vi "LaneFolower.vi"() -> ()   [LabVIEW 2024]
uses:
  <vilib>/Python/Open Venv Python Session.vi
panel:
  in  "File Path":path
  out "Image":T1(plugin-control)
  in  "Lane_No.":i32
  out "ToGoLane_X":dbl[](array[numeric])=[-0.07318960875272751, -0.07601258158683777, -0.07903728634119034, -0.08227015286684036, -0.08571790158748627, -0.08938748389482498, -0.09328625351190567, -0.09742185473442078, -0.1018022671341896, -0.10643591731786728, -0.11133154481649399, -0.11649835854768753, -0.12194599956274033, -0.1276845932006836, -0.13372473418712616, -0.140077605843544, -0.1467549204826355, -0.15376901626586914, -0.1611328274011612, -0.16886006295681, -0.17696507275104523, -0.18546302616596222, -0.19436998665332794, -0.20370280742645264, -0.2134794145822525, -0.22371862828731537, -0.23444052040576935, -0.2456662356853485, -0.2574182152748108, -0.26972031593322754, -0.2825978398323059, -0.2960776686668396, -0.3101884424686432, -0.3249606192111969, -0.3404266834259033, -0.35662132501602173, -0.3735816180706024, -0.39134714007377625, -0.4099603295326233, -0.4294666647911072, -0.44991496205329895, -0.47135770320892334, -0.49385130405426025, -0.5174566507339478, -0.5422393083572388, -0.5682703852653503, -0.5956265330314636, -0.6243910789489746, -0.6546544432640076, -0.6865149736404419]
  out "ToGpLane_Y":dbl[](array[numeric])=[0.040495745837688446, 0.047222185879945755, 0.05409690737724304, 0.06112465262413025, 0.06831060349941254, 0.07565993815660477, 0.08317827433347702, 0.09087134152650833, 0.09874525666236877, 0.10680633038282394, 0.1150611862540245, 0.12351679056882858, 0.13218039274215698, 0.14105971157550812, 0.1501627415418625, 0.159497931599617, 0.16907407343387604, 0.1789005994796753, 0.18898724019527435, 0.19934435188770294, 0.20998279750347137, 0.22091402113437653, 0.23215018212795258, 0.24370405077934265, 0.2555891275405884, 0.2678196132183075, 0.2804107666015625, 0.2933785319328308, 0.306739866733551, 0.3205127418041229, 0.3347163796424866, 0.349371075630188, 0.36449843645095825, 0.38012149930000305, 0.3962647616863251, 0.41295456886291504, 0.43021881580352783, 0.4480874836444855, 0.46659258008003235, 0.48576855659484863, 0.5056522488594055, 0.526283323764801, 0.5477043986320496, 0.5699615478515625, 0.5931042432785034, 0.6171862483024597, 0.6422654986381531, 0.6684049367904663, 0.6956729292869568, 0.7241437435150146]
  out "Tracking_Err(m)":dbl=0.08364582631744388
  in  "Ld(m)":dbl=1.0 format="%#_13g"
  out "GPS_Steer_CMD(Deg)":dbl=-20.0
  out "Lane":T2(graph)=[{"Third_Lane_X"=[-0.07318960875272751, -0.07601258158683777, -0.07903728634119034, -0.08227015286684036, -0.08571790158748627, -0.08938748389482498, -0.09328625351190567, -0.09742185473442078, -0.1018022671341896, -0.10643591731786728, -0.11133154481649399, -0.11649835854768753, -0.12194599956274033, -0.1276845932006836, -0.13372473418712616, -0.140077605843544, -0.1467549204826355, -0.15376901626586914, -0.1611328274011612, -0.16886006295681, -0.17696507275104523, -0.18546302616596222, -0.19436998665332794, -0.20370280742645264, -0.2134794145822525, -0.22371862828731537, -0.23444052040576935, -0.2456662356853485, -0.2574182152748108, -0.26972031593322754, -0.2825978398323059, -0.2960776686668396, -0.3101884424686432, -0.3249606192111969, -0.3404266834259033, -0.35662132501602173, -0.3735816180706024, -0.39134714007377625, -0.4099603295326233, -0.4294666647911072, -0.44991496205329895, -0.47135770320892334, -0.49385130405426025, -0.5174566507339478, -0.5422393083572388, -0.5682703852653503, -0.5956265330314636, -0.6243910789489746, -0.6546544432640076, -0.6865149736404419], "Third_Lane_Y"=[0.040495745837688446, 0.047222185879945755, 0.05409690737724304, 0.06112465262413025, 0.06831060349941254, 0.07565993815660477, 0.08317827433347702, 0.09087134152650833, 0.09874525666236877, 0.10680633038282394, 0.1150611862540245, 0.12351679056882858, 0.13218039274215698, 0.14105971157550812, 0.1501627415418625, 0.159497931599617, 0.16907407343387604, 0.1789005994796753, 0.18898724019527435, 0.19934435188770294, 0.20998279750347137, 0.22091402113437653, 0.23215018212795258, 0.24370405077934265, 0.2555891275405884, 0.2678196132183075, 0.2804107666015625, 0.2933785319328308, 0.306739866733551, 0.3205127418041229, 0.3347163796424866, 0.349371075630188, 0.36449843645095825, 0.38012149930000305, 0.3962647616863251, 0.41295456886291504, 0.43021881580352783, 0.4480874836444855, 0.46659258008003235, 0.48576855659484863, 0.5056522488594055, 0.526283323764801, 0.5477043986320496, 0.5699615478515625, 0.5931042432785034, 0.6171862483024597, 0.6422654986381531, 0.6684049367904663, 0.6956729292869568, 0.7241437435150146]}, {"Third_Lane_X"=[0.3850393295288086, 0.38269442319869995, 0.3802776634693146, 0.37778156995773315, 0.37519851326942444, 0.37252023816108704, 0.36973854899406433, 0.3668445944786072, 0.36382946372032166, 0.3606834411621094, 0.3573968708515167, 0.35395947098731995, 0.3503605127334595, 0.3465888500213623, 0.34263283014297485, 0.3384802043437958, 0.33411839604377747, 0.3295340836048126, 0.3247132897377014, 0.31964147090911865, 0.3143034875392914, 0.3086833655834198, 0.30276429653167725, 0.29652881622314453, 0.2899583876132965, 0.2830337584018707, 0.2757345139980316, 0.2680392861366272, 0.2599255442619324, 0.25136950612068176, 0.24234625697135925, 0.23282931745052338, 0.22279086709022522, 0.21220147609710693, 0.201029971241951, 0.1892433911561966, 0.17680683732032776, 0.16368332505226135, 0.14983347058296204, 0.135215625166893, 0.1197853684425354, 0.10349543392658234, 0.0862954780459404, 0.06813178956508636, 0.048946939408779144, 0.028679724782705307, 0.007264426909387112, -0.015369318425655365, -0.03929702565073967, -0.06459984183311462], "Third_Lane_Y"=[0.07649079710245132, 0.08298972249031067, 0.08961328864097595, 0.09636534750461578, 0.10325001180171967, 0.11027147620916367, 0.11743411421775818, 0.12474247813224792, 0.1322014033794403, 0.1398158222436905, 0.14759093523025513, 0.155532106757164, 0.16364507377147675, 0.17193572223186493, 0.180410236120224, 0.18907500803470612, 0.19793690741062164, 0.20700296759605408, 0.21628059446811676, 0.2257775366306305, 0.23550201952457428, 0.2454625517129898, 0.25566813349723816, 0.2661281228065491, 0.276852548122406, 0.28785181045532227, 0.29913684725761414, 0.31071919202804565, 0.32261112332344055, 0.33482545614242554, 0.3473757207393646, 0.3602762222290039, 0.3735422194004059, 0.387189656496048, 0.4012354910373688, 0.4156976342201233, 0.4305952489376068, 0.4459485411643982, 0.4617789089679718, 0.4781092703342438, 0.4949638843536377, 0.5123687386512756, 0.5303513407707214, 0.5489413142204285, 0.5681700706481934, 0.5880714654922485, 0.6086814403533936, 0.6300389170646667, 0.6521854400634766, 0.6751657128334045]}, {"Third_Lane_X"=[0.0, 0.0, 0.0, 0.0, 0.0, 0.0, 0.0, 0.0, 0.0, 0.0, 0.0, 0.0, 0.0, 0.0, 0.0, 0.0, 0.0, 0.0, 0.0, 0.0, 0.0, 0.0, 0.0, 0.0, 0.0, 0.0, 0.0, 0.0, 0.0, 0.0, 0.0, 0.0, 0.0, 0.0, 0.0, 0.0, 0.0, 0.0, 0.0, 0.0, 0.0, 0.0, 0.0, 0.0, 0.0, 0.0, 0.0, 0.0, 0.0, 0.0], "Third_Lane_Y"=[0.0, 0.0, 0.0, 0.0, 0.0, 0.0, 0.0, 0.0, 0.0, 0.0, 0.0, 0.0, 0.0, 0.0, 0.0, 0.0, 0.0, 0.0, 0.0, 0.0, 0.0, 0.0, 0.0, 0.0, 0.0, 0.0, 0.0, 0.0, 0.0, 0.0, 0.0, 0.0, 0.0, 0.0, 0.0, 0.0, 0.0, 0.0, 0.0, 0.0, 0.0, 0.0, 0.0, 0.0, 0.0, 0.0, 0.0, 0.0, 0.0, 0.0]}]
  out "Third_Lane_X":dbl[](array[numeric])
  out "Third_Lane_Y":dbl[](array[numeric])
  out "Second_Lane_X":dbl[](array[numeric])=[0.3850393295288086, 0.38269442319869995, 0.3802776634693146, 0.37778156995773315, 0.37519851326942444, 0.37252023816108704, 0.36973854899406433, 0.3668445944786072, 0.36382946372032166, 0.3606834411621094, 0.3573968708515167, 0.35395947098731995, 0.3503605127334595, 0.3465888500213623, 0.34263283014297485, 0.3384802043437958, 0.33411839604377747, 0.3295340836048126, 0.3247132897377014, 0.31964147090911865, 0.3143034875392914, 0.3086833655834198, 0.30276429653167725, 0.29652881622314453, 0.2899583876132965, 0.2830337584018707, 0.2757345139980316, 0.2680392861366272, 0.2599255442619324, 0.25136950612068176, 0.24234625697135925, 0.23282931745052338, 0.22279086709022522, 0.21220147609710693, 0.201029971241951, 0.1892433911561966, 0.17680683732032776, 0.16368332505226135, 0.14983347058296204, 0.135215625166893, 0.1197853684425354, 0.10349543392658234, 0.0862954780459404, 0.06813178956508636, 0.048946939408779144, 0.028679724782705307, 0.007264426909387112, -0.015369318425655365, -0.03929702565073967, -0.06459984183311462]
  out "Second_Lane_Y":dbl[](array[numeric])=[0.07649079710245132, 0.08298972249031067, 0.08961328864097595, 0.09636534750461578, 0.10325001180171967, 0.11027147620916367, 0.11743411421775818, 0.12474247813224792, 0.1322014033794403, 0.1398158222436905, 0.14759093523025513, 0.155532106757164, 0.16364507377147675, 0.17193572223186493, 0.180410236120224, 0.18907500803470612, 0.19793690741062164, 0.20700296759605408, 0.21628059446811676, 0.2257775366306305, 0.23550201952457428, 0.2454625517129898, 0.25566813349723816, 0.2661281228065491, 0.276852548122406, 0.28785181045532227, 0.29913684725761414, 0.31071919202804565, 0.32261112332344055, 0.33482545614242554, 0.3473757207393646, 0.3602762222290039, 0.3735422194004059, 0.387189656496048, 0.4012354910373688, 0.4156976342201233, 0.4305952489376068, 0.4459485411643982, 0.4617789089679718, 0.4781092703342438, 0.4949638843536377, 0.5123687386512756, 0.5303513407707214, 0.5489413142204285, 0.5681700706481934, 0.5880714654922485, 0.6086814403533936, 0.6300389170646667, 0.6521854400634766, 0.6751657128334045]
  out "First_Lane_Y":dbl[](array[numeric])=[0.040495745837688446, 0.047222185879945755, 0.05409690737724304, 0.06112465262413025, 0.06831060349941254, 0.07565993815660477, 0.08317827433347702, 0.09087134152650833, 0.09874525666236877, 0.10680633038282394, 0.1150611862540245, 0.12351679056882858, 0.13218039274215698, 0.14105971157550812, 0.1501627415418625, 0.159497931599617, 0.16907407343387604, 0.1789005994796753, 0.18898724019527435, 0.19934435188770294, 0.20998279750347137, 0.22091402113437653, 0.23215018212795258, 0.24370405077934265, 0.2555891275405884, 0.2678196132183075, 0.2804107666015625, 0.2933785319328308, 0.306739866733551, 0.3205127418041229, 0.3347163796424866, 0.349371075630188, 0.36449843645095825, 0.38012149930000305, 0.3962647616863251, 0.41295456886291504, 0.43021881580352783, 0.4480874836444855, 0.46659258008003235, 0.48576855659484863, 0.5056522488594055, 0.526283323764801, 0.5477043986320496, 0.5699615478515625, 0.5931042432785034, 0.6171862483024597, 0.6422654986381531, 0.6684049367904663, 0.6956729292869568, 0.7241437435150146]
  out "First_Lane_X":dbl[](array[numeric])=[-0.07318960875272751, -0.07601258158683777, -0.07903728634119034, -0.08227015286684036, -0.08571790158748627, -0.08938748389482498, -0.09328625351190567, -0.09742185473442078, -0.1018022671341896, -0.10643591731786728, -0.11133154481649399, -0.11649835854768753, -0.12194599956274033, -0.1276845932006836, -0.13372473418712616, -0.140077605843544, -0.1467549204826355, -0.15376901626586914, -0.1611328274011612, -0.16886006295681, -0.17696507275104523, -0.18546302616596222, -0.19436998665332794, -0.20370280742645264, -0.2134794145822525, -0.22371862828731537, -0.23444052040576935, -0.2456662356853485, -0.2574182152748108, -0.26972031593322754, -0.2825978398323059, -0.2960776686668396, -0.3101884424686432, -0.3249606192111969, -0.3404266834259033, -0.35662132501602173, -0.3735816180706024, -0.39134714007377625, -0.4099603295326233, -0.4294666647911072, -0.44991496205329895, -0.47135770320892334, -0.49385130405426025, -0.5174566507339478, -0.5422393083572388, -0.5682703852653503, -0.5956265330314636, -0.6243910789489746, -0.6546544432640076, -0.6865149736404419]
  out "error out":errorcluster
  out "Python Loop Process Time":u32=34
  in  "stop":bool
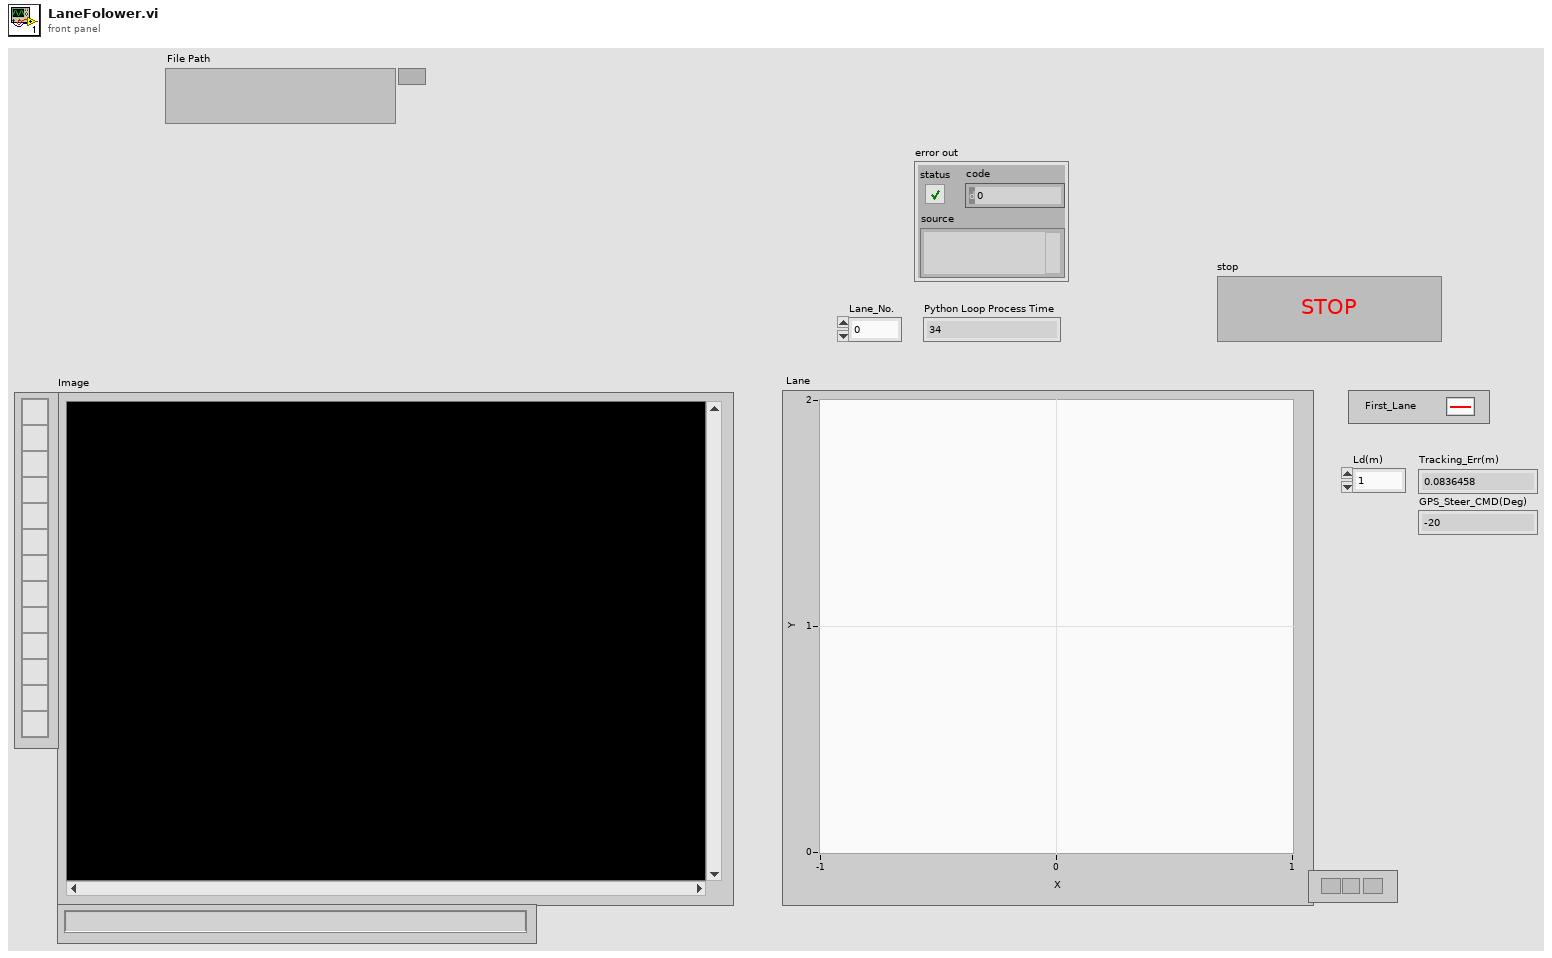
[diagram p1: front panel]
types:
  T1 = typedef "IMAQ Image.ctl" = refnum<image>
  T2 = cluster{"Third_Lane_X":dbl[], "Third_Lane_Y":dbl[]}[]
  T3 = cluster{"First_Lane_X":dbl[], "First_Lane_Y":dbl[]}
  T4 = cluster{"Second_Lane_X":dbl[], "Second_Lane_Y":dbl[]}
  T5 = cluster{"Third_Lane_X":dbl[], "Third_Lane_Y":dbl[]}
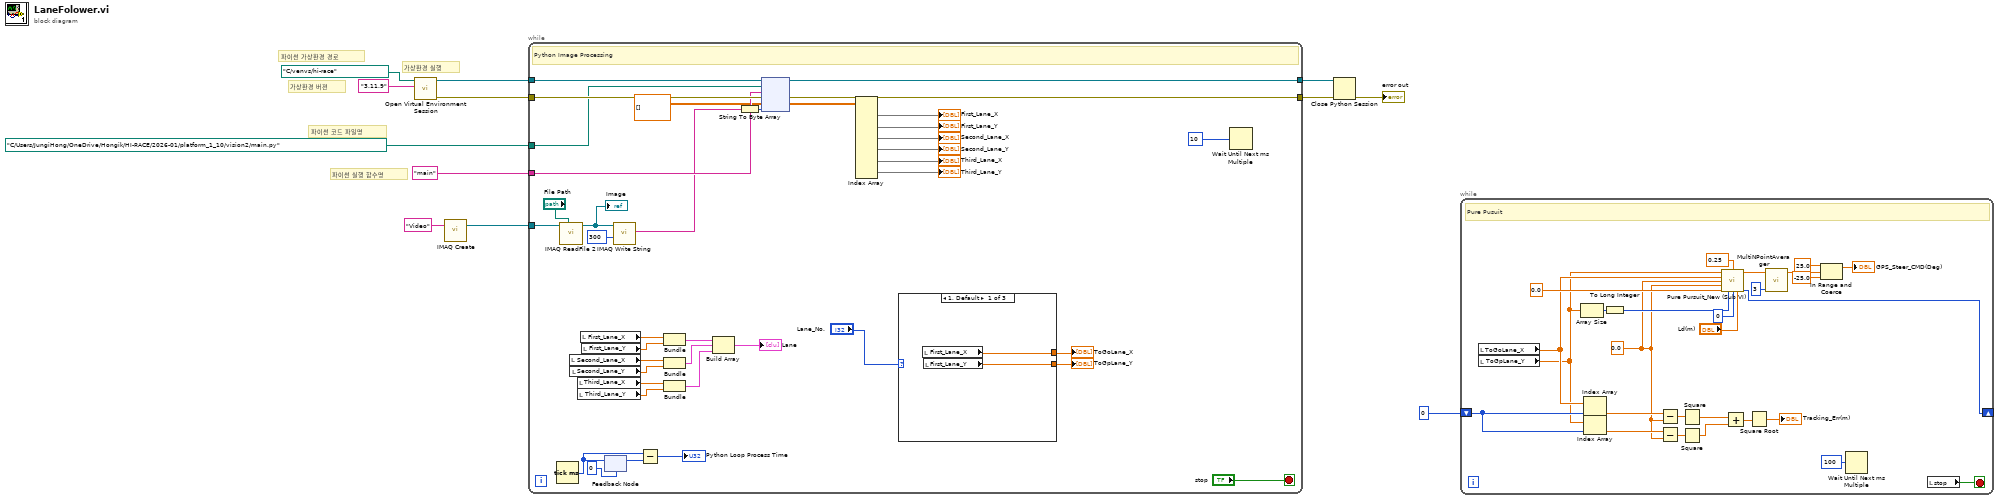
[diagram p0: block diagram]
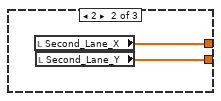
[diagram p2: hidden frame]
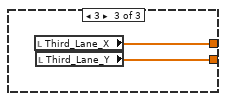
[diagram p3: hidden frame]
diagram:
  # "파이썬 실행 함수명"
  # "파이썬 코드 파일명"
  # "가상환경 실행"
  # "가상환경 버젼"
  # "파이썬 가상환경 경로"
  n1 = call-poly <vilib>:"Open Virtual Environment Session.vi"("Python version"="3.11.9", "Env path"=path "C:/venvs/hi-race") -> ("error out"=w7:errorcluster, "session out"=w8:refnum<k35>)  [unwired: 8 in]
  n2 = call "IMAQ Create"("Image Name"="Video") -> ("New Image"=w1:T1)  [unwired: 4 in, 1 out]
  n3 = while {
    tunnel: path "C:/Users/JungiHong/OneDrive/Hongik/HI-RACE/2026-01/platform_1_10/vision2/main.py" ("Name") -> [w47]
    tunnel: "main" ("module out") -> [w46]
    tunnel: w8 -> [w49]
    tunnel: [w51] -> w10
    tunnel: w7 -> [w48]
    tunnel: [w50] -> w9
    tunnel: w1 -> [w15]
    stop <- "stop" stop-if-true
    # "Python Image Processing"
    n4 = Tick Count (ms)() -> (millisecond timer value=w42:u32)
    n5 = call "IMAQ ReadFile 2"("File Path"="File Path", "Image"=w15) -> ("Image Out"=w14:T1)  [unwired: 5 in, 4 out]
    "Image" <- w14
    n6 = local read "Second_Lane_X"() -> (w32:dbl[])
    n7 = local read "Second_Lane_Y"() -> (w31:dbl[])
    n8 = local read "Third_Lane_X"() -> (w30:dbl[])
    n9 = local read "Third_Lane_Y"() -> (w29:dbl[])
    n10 = local read "First_Lane_X"() -> (w34:dbl[])
    n11 = local read "First_Lane_Y"() -> (w33:dbl[])
    n12 = feedback #1(u32 0 ("millisecond timer value")) -> (w43:u32)
    n13 = feedback-in #1(w42) -> ()
    n14 = call-poly "IMAQ Write String"("Image Quality"=u32 300, "Image"=w14) -> ("FileString"=w16:string)  [unwired: 7 in, 2 out]
    n15 = Subtract(x=w42, y=w43) -> (x-y=→"Python Loop Process Time":u32)
    n16 = Bundle("First_Lane_X"=w34, "First_Lane_Y"=w33) -> (w28:T3)  [unwired: 1 in]
    n17 = Bundle("Second_Lane_X"=w32, "Second_Lane_Y"=w31) -> (w27:T4)  [unwired: 1 in]
    n18 = Bundle("Third_Lane_X"=w30, "Third_Lane_Y"=w29) -> (w26:T5)  [unwired: 1 in]
    n19 = Build Array(w28, w27, w26) -> (→"Lane":T2)
    n20 = String To Byte Array(string=w16) -> (unsigned byte array=w41:u8[])
    n21 = node(w49, w47, w46, w48, dbl[][] [] ("appended array"), w41) -> (w51:refnum<k35>, w50:errorcluster, w20:dbl[][])  [unwired: 1 in, 2 out]
    n22 = Index Array(array=w20) -> (element #1=→"First_Lane_X":dbl[], element #2=→"First_Lane_Y":dbl[], element #3=→"Second_Lane_X":dbl[], element #4=→"Second_Lane_Y":dbl[], element #5=→"Third_Lane_X":dbl[], element #6=→"Third_Lane_Y":dbl[])  [unwired: 12 in]
    n23 = case shown="1, Default" "Lane_No." {
      tunnel: [w53 w55 w57] -> w23
      tunnel: [w52 w54 w56] -> w22
      frame 1, Default {
        n24 = local read "First_Lane_X"() -> (w53:dbl[])
        n25 = local read "First_Lane_Y"() -> (w52:dbl[])
      }
      frame 2 {
        n26 = local read "Second_Lane_X"() -> (w55:dbl[])
        n27 = local read "Second_Lane_Y"() -> (w54:dbl[])
      }
      frame 3 {
        n28 = local read "Third_Lane_X"() -> (w57:dbl[])
        n29 = local read "Third_Lane_Y"() -> (w56:dbl[])
      }
    }
    "ToGoLane_X" <- w23
    "ToGpLane_Y" <- w22
    n30 = Wait Until Next ms Multiple(millisecond multiple=u32 10) -> ()  [unwired: 1 out]
  }
  n31 = Close Python Session(session in=w10, error in=w9) -> (11:→"error out":errorcluster)
  n32 = while {
    shift-right: [w84] -> _
    shift-left: 0 ("Index(near vehicle)") -> [w83]
    stop <- w82 stop-if-true
    w58 = 0.0 ("Y_Current")
    # "Pure Pusuit"
    n33 = local read "ToGoLane_X"() -> (w60:dbl[])
    n34 = local read "ToGpLane_Y"() -> (w59:dbl[])
    n35 = Array Size(array=w59) -> (size(s)=w69:i32)
    n36 = Index Array(array=w60, index=w83) -> (element=w80:dbl)
    n37 = Index Array(array=w59, index=w83) -> (element=w81:dbl)
    n38 = To Long Integer(number=w69) -> (32bit integer=w68:i32)
    n39 = Subtract(x=w80, y=w58) -> (x-y=w75:dbl)
    n40 = Subtract(x=w81, y=w58) -> (x-y=w74:dbl)
    n41 = Square(x=w75) -> (x^2=w73:dbl)
    n42 = Square(x=w74) -> (x^2=w72:dbl)
    n43 = call "Pure Pursuit_New (Sub VI).vi"("x_lat_path"=w59, "L"=0.25, "y_long_path"=w60, "X_Current"=w58, "Y_Current"=w58, "Heading_Current"=0.0, "#pnt"=w68, "WP no_pre"=0, "LAD"="Ld(m)") -> ("Steer_CMD(Deg)"=w64:dbl, "Index(near vehicle)"=w84:i32)  [unwired: 3 in, 2 out]
    n44 = Add(x=w73, y=w72) -> (x+y=w71:dbl)
    n45 = Square Root(x=w71) -> (sqrt(x)=→"Tracking_Err(m)":dbl)
    n46 = call "MultiNPointAverager.vi"("N point average"=3 ("WP no_pre"), "Data_input"=w64) -> ("숫자형"=w79:dbl)  [unwired: 9 in]
    n47 = In Range and Coerce(upper limit=25.0, x=w79, lower limit=-25.0) -> (coerced(x)=→"GPS_Steer_CMD(Deg)":dbl)  [unwired: 1 out]
    n48 = Wait Until Next ms Multiple(millisecond multiple=u32 100 ("ms 배수")) -> ()  [unwired: 1 out]
    n49 = local read "stop"() -> (w82:bool)
  }
